vi "_Standardize Carriage Returns.vi"(11 "States":string) -> (3 "trimed text":string)   [LabVIEW 2017, in "csmdoc.lvlib"]
uses:
  csmdoc.lvlib
  _Shared/CSM Shared.lvlib
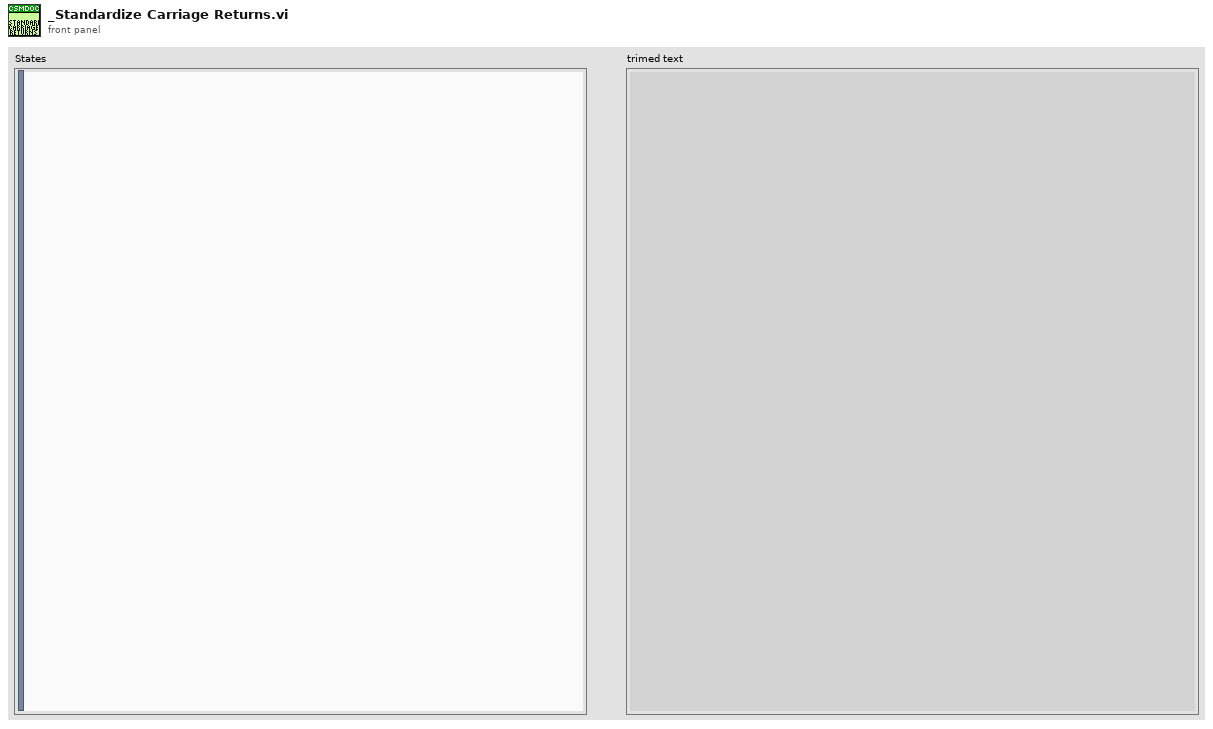
[diagram p1: front panel]
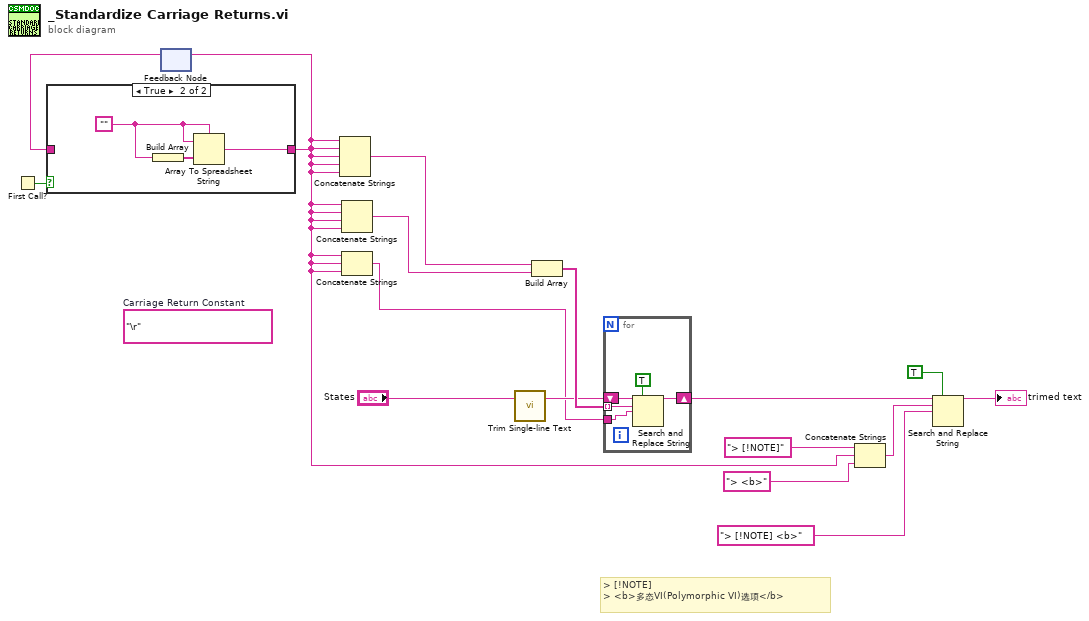
[diagram p0: block diagram]
diagram:
  (unwired) "\r"  # Carriage Return Constant
  # "> [!NOTE]\n> <b>多态VI(Polymorphic VI)选项</b>"
  n1 = First Call?() -> (First Call?: T/F=w13:bool)
  n2 = feedback #1() -> (w14:string)  [unwired: 1 in]
  n3 = case shown="True" w13 {
    tunnel: [w17 w18] -> w2
    tunnel: w14 -> [w17 _]
    frame False {
    }
    frame True {
      w19 = "" ("Empty String\n(hidden on FP)")
      n4 = Build Array(w19) -> (w20:string[])
      n5 = Array To Spreadsheet String(delimiter (Tab)=w19, array=w20, 3:w19) -> (spreadsheet string=w18:string)
    }
  }
  n6 = feedback-in #1(w2) -> ()
  n7 = Concatenate Strings(w2, w2, w2, w2, w2) -> (w15:string)
  n8 = Concatenate Strings(w2, w2, w2, w2) -> (w16:string)
  n9 = Concatenate Strings(w2, w2, w2) -> (w10:string)
  n10 = call "Trim Single-line Text.vi"("single-line text"="States") -> ("trimed text"=w11:string)  [unwired: 2 in]
  n11 = Build Array(w15, w16) -> (w12:string[])
  n12 = for {
    shift-right: [w25] -> w9
    shift-left: w11 -> [w24]
    tunnel: w12 -> [w22] mode=indexing
    tunnel: w10 -> [w21]
    n13 = Search and Replace String(replace all?=TRUE ("replace all? (F)"), input string=w24, search string=w22, replace string=w21) -> (result string=w25:string)  [unwired: 4 in, 3 out]
  }
  n14 = Concatenate Strings("> [!NOTE]" ("search string"), w2, "> <b>" ("search string")) -> (w5:string)
  n15 = Search and Replace String(replace all?=TRUE ("replace all? (F)"), input string=w9, search string=w5, replace string="> [!NOTE] <b>" ("search string")) -> (result string=→"trimed text":string)  [unwired: 4 in, 3 out]
